vi "FileStream Initialize.vi"(8 "error in (no error)":errorcluster, 9 "mode":i32(ring)=1 items=["CreateNew"=1, "Create"=2, "Open"=3, "OpenOrCreate"=4, "Truncate"=5, "Append"=6], 11 "path":path) -> (0 "error out":errorcluster, 3 "new reference":refnum<k24>)   [LabVIEW 2017, in "File Stream.lvlib"]
doc: "Initializes a new instance of the FileStream class with the specified path and creation mode."
uses:
  File Stream.lvlib
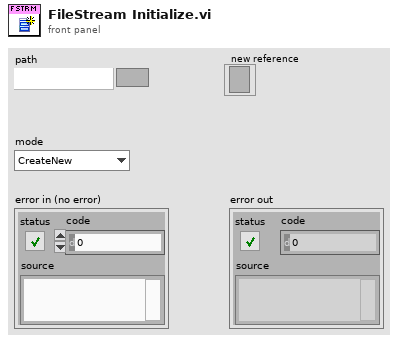
[diagram p1: front panel]
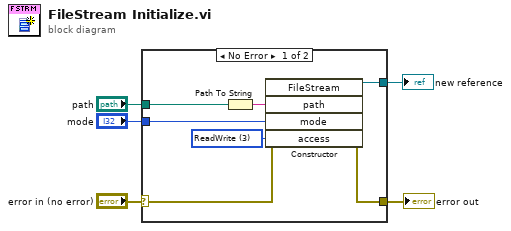
[diagram p0: block diagram]
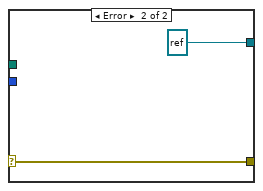
[diagram p2: hidden frame]
diagram:
  n1 = case shown="No Error" "error in (no error)" {
    selector: "error in (no error)" -> [w9 w14]
    tunnel: "mode" -> [w11 _]
    tunnel: "path" -> [w10 _]
    tunnel: [w8 refnum<k24> refnum ("new reference")] -> w2
    tunnel: [w7 w14] -> w1
    frame No Error {
      w6 = 3 items=["Read"=1, "Write"=2, "ReadWrite"=3] ("access")
      n2 = Path To String(path=w10) -> (string=w12:string)
      n3 = constructor class="FileStream"(error in=w9, "path"=w12, "mode"=w11, "access"=w6) -> (reference out=w8:refnum<k24>, error out=w7:errorcluster)  [unwired: 2 in, 4 out]
    }
    frame Error {
    }
  }
  "new reference" <- w2
  "error out" <- w1
